vi "Set All Plot Visibility (WFChart).vi"(8 "error in (no error)":errorcluster, 10 "All Visible?":bool, 11 "WaveformChart in":refnum<vi>) -> (0 "error out":errorcluster, 3 "WaveformChart out":refnum<vi>)   [LabVIEW 2019, in "Instrument.Lockin.lvlib" / "Instrument UI.Lockin.lvclass"]
uses:
  Instrument UI.Lockin.lvclass
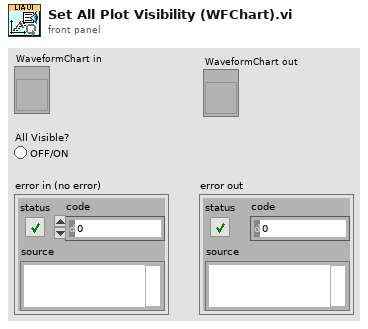
[diagram p1: front panel]
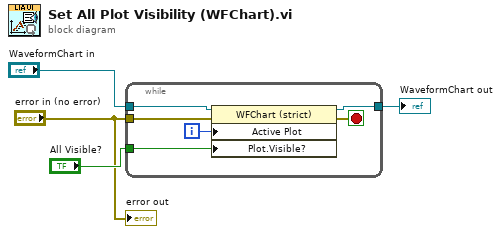
[diagram p0: block diagram]
diagram:
  n1 = while {
    tunnel: "WaveformChart in" -> [w6]
    tunnel: "error in (no error)" -> [w7]
    tunnel: [w10] -> w2
    tunnel: "All Visible?" -> [w8]
    i -> [w9]
    stop <- w5 stop-if-true
    n2 = property on="Property Node" class="WFChart (strict)"(reference=w6, error in=w7, "Active Plot"=w9, "Plot.Visible?"=w8) -> (reference out=w10:refnum<vi>, error out=w5:errorcluster)
  }
  "WaveformChart out" <- w2
  "error out" <- "error in (no error)"
